vi "TestMethod.vi"() -> ()   [LabVIEW 2015]
panel:
  out "数据缓存":u8[](array[numeric])
  in  "停止":bool
  out "波形图":sgl[](graph)
  in  "读取方式":enum16{"bin", "csv"}(ring)
  in  "抓取波形数据指令集合":string(combo)="capture wave:.bin@CH:0@DT:vol;"
  out "Dll路径":path
  in  "超时(ms)":u32=2000
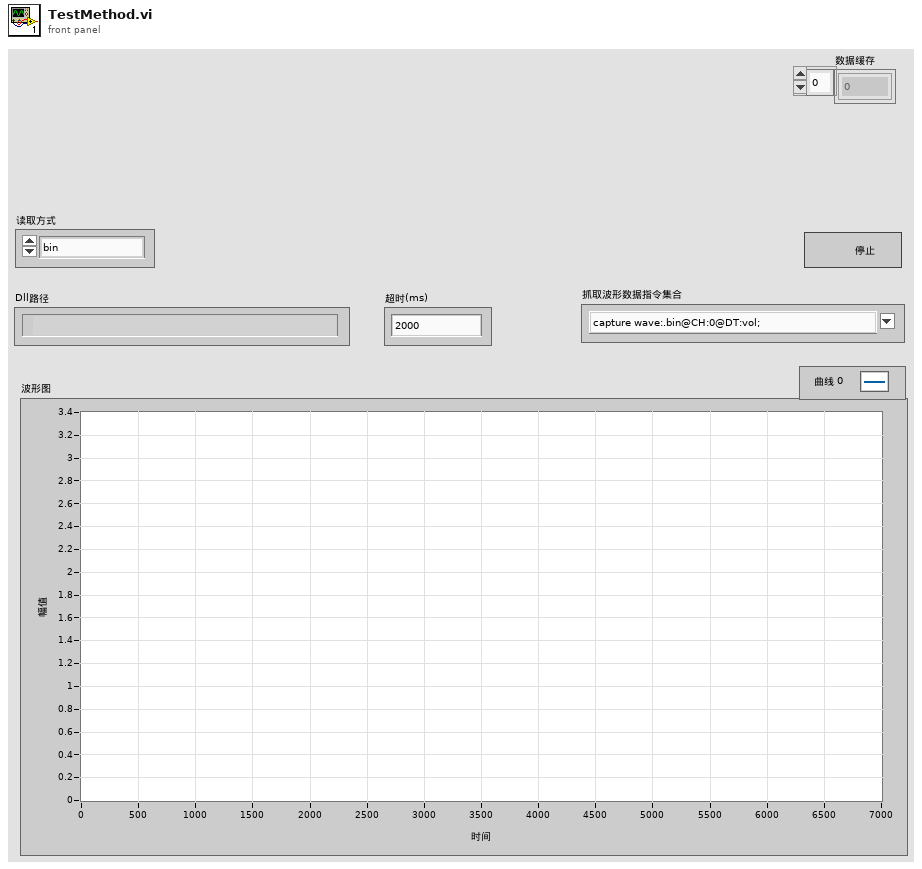
[diagram p1: front panel]
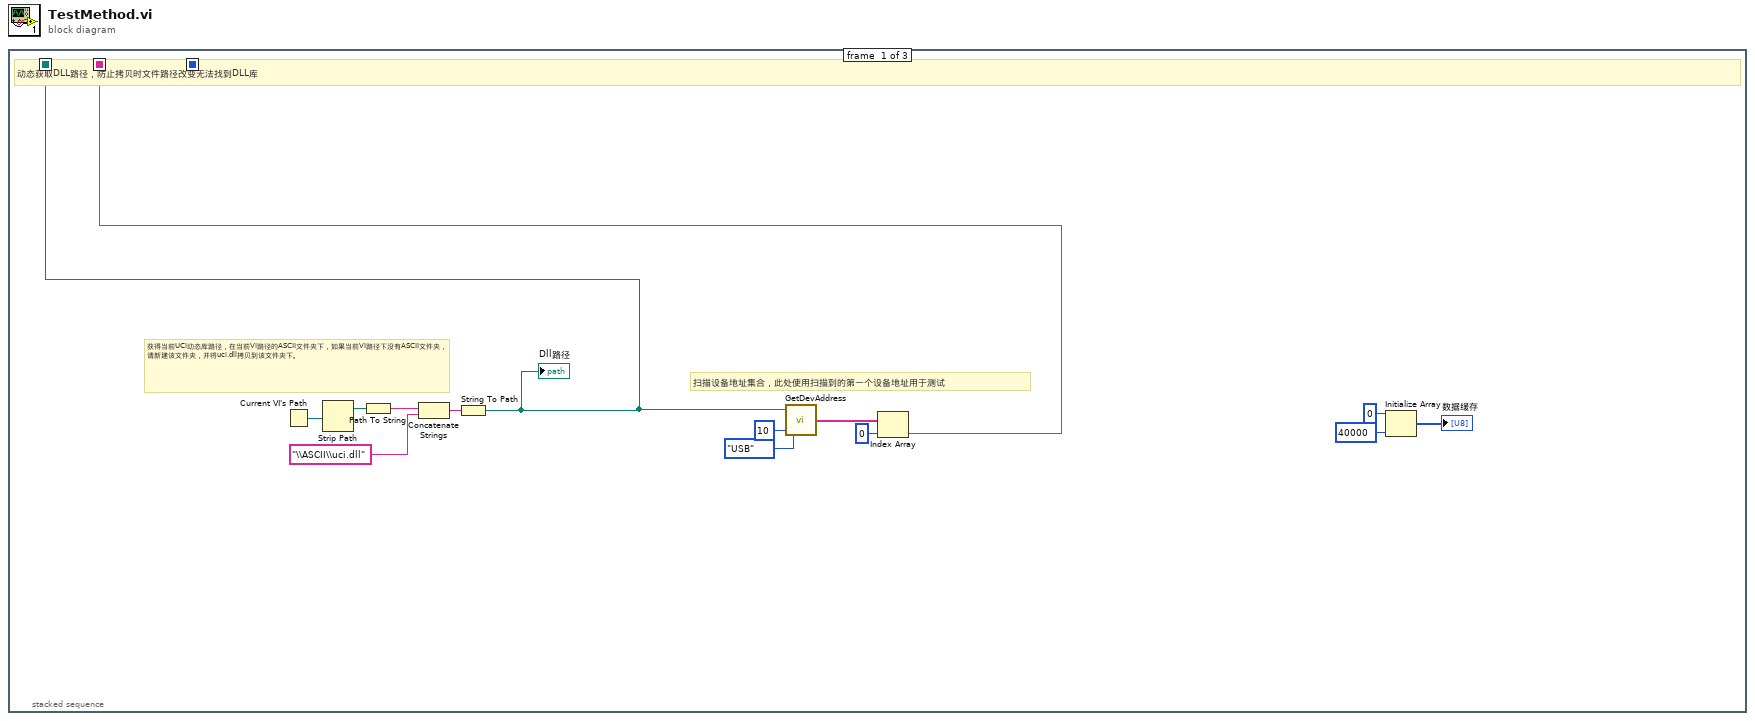
[diagram p0: block diagram]
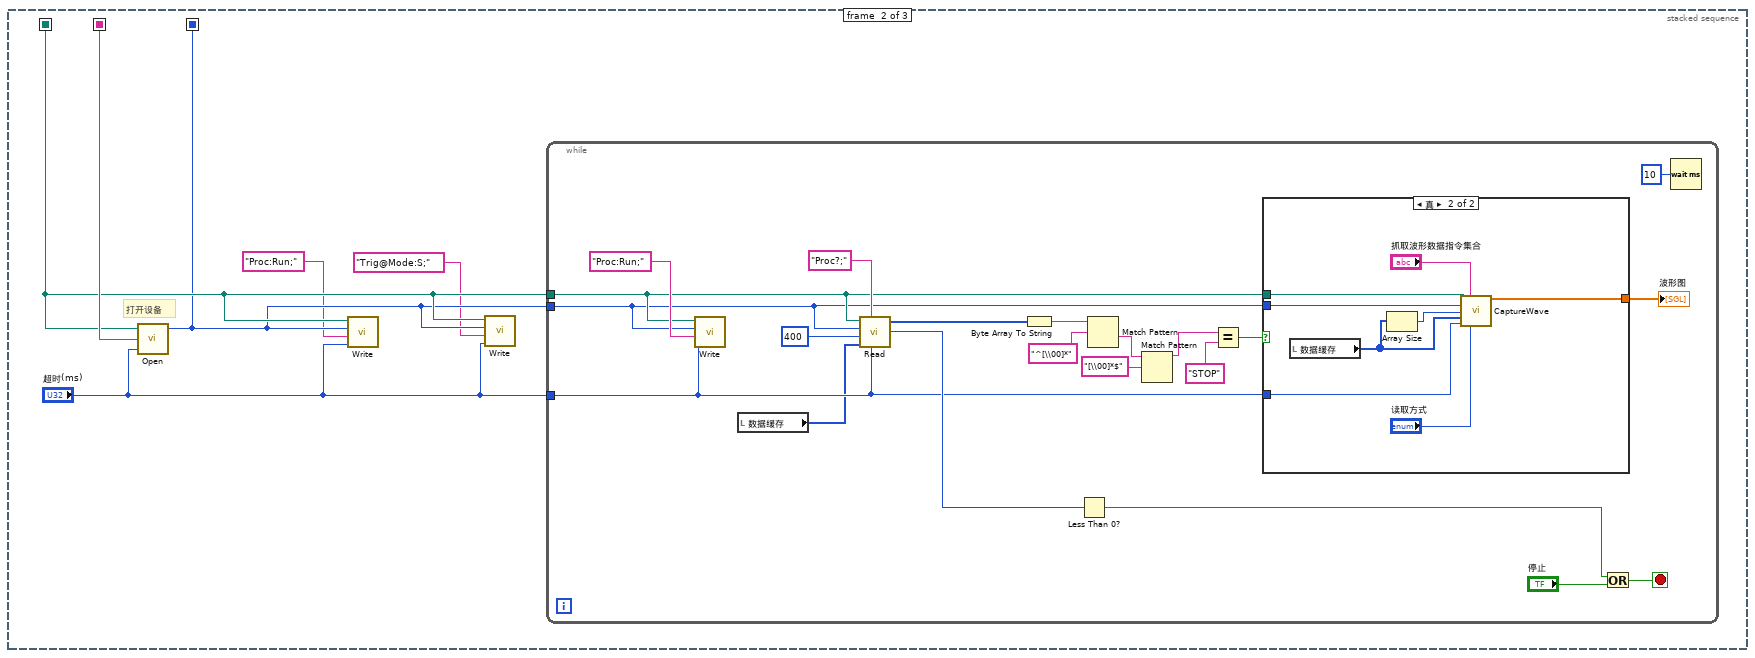
[diagram p2: hidden frame]
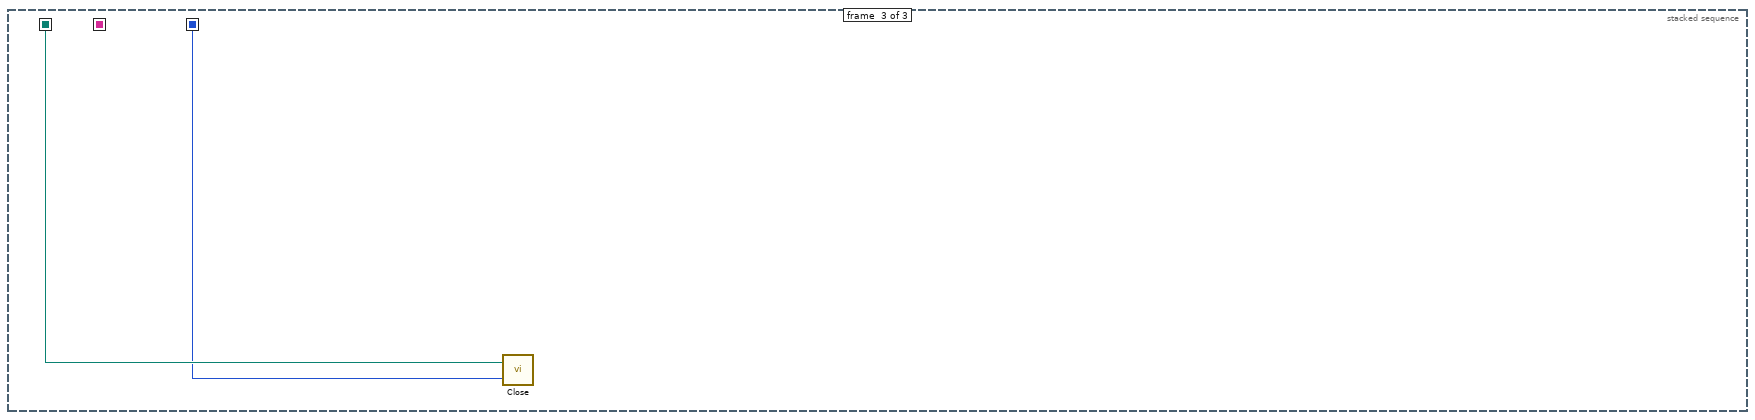
[diagram p4: hidden frame]
diagram:
  n1 = stacked-sequence {
    seq-local: [w9 _ _] -> [_ w19 w51]
    seq-local: [_ w18 _] -> [_ _ w50]
    seq-local: [w4 _ _] -> [_ w20 _]
    frame #0 {
      # "扫描设备地址集合，此处使用扫描到的第一个设备地址用于测试"
      # "获得当前UCI动态库路径，在当前VI路径的ASCII文件夹下，如果当前VI路径下没有ASCII文件夹，请新建该文件夹，并将uci.dll拷贝到该文件夹下。"
      # "动态获取DLL路径，防止拷贝时文件路径改变无法找到DLL库"
      n2 = Current VI's Path() -> (path=w13:path)
      n3 = Strip Path(path=w13) -> (stripped path=w11:path)  [unwired: 1 out]
      n4 = Path To String(path=w11) -> (string=w10:string)
      n5 = Concatenate Strings(w10, "\\ASCII\\uci.dll" ("字符串")) -> (w12:string)
      n6 = String To Path(string=w12) -> (path=w9:path)
      "Dll路径" <- w9
      n7 = call "GetDevAddress.vi"("DevNum"=u32 10 ("搜索设备数量"), "DevType"=enum16{"LAN", "USB"}."USB" ("设备类型"), "UCI_DllPath"=w9) -> ("DevAddressGroup"=w6:string[])
      n8 = Index Array(array=w6, index=0 ("索引")) -> (element=w4:string)
      n9 = Initialize Array(u8 0 ("元素"), 40000 ("维数大小")) -> (→"数据缓存":u8[])
    }
    frame #1 {
      # "打开设备"
      n10 = call "Open.vi"("Timeout"="超时(ms)", "Addr"=w20, "UCI_DllPath"=w19) -> ("Session_id"=w18:i32)  [unwired: 2 out]
      n11 = call "Write.vi"("UCI_DllPath"=w19, "Session_id"=w18, "Command"="Proc:Run;" ("指令"), "Timeout"="超时(ms)") -> ()  [unwired: 1 in, 1 out]
      n12 = call "Write.vi"("UCI_DllPath"=w19, "Session_id"=w18, "Command"="Trig@Mode:S;" ("指令"), "Timeout"="超时(ms)") -> ()  [unwired: 1 in, 1 out]
      n13 = while {
        tunnel: w19 -> [w29]
        tunnel: w18 -> [w27]
        tunnel: "超时(ms)" -> [w28]
        stop <- w24 stop-if-true
        n14 = call "Write.vi"("UCI_DllPath"=w29, "Session_id"=w27, "Command"="Proc:Run;" ("指令"), "Timeout"=w28) -> ()  [unwired: 1 in, 1 out]
        n15 = local read "数据缓存"() -> (w22:u8[])
        n16 = call "Read.vi"("UCI_DllPath"=w29, "Command"="Proc?;" ("指令"), "Session_id"=w27, "Length"=u32 400 ("len"), "Timeout"=w28, "InputData"=w22) -> ("OutputData"=w40:u8[], "Result"=w33:i32)  [unwired: 1 out]
        n17 = Byte Array To String(unsigned byte array=w40) -> (string=w34:string)
        n18 = Less Than 0?(x=w33) -> (x < 0?=w23:bool)
        n19 = Match Pattern(string=w34, regular expression="^[\\00]*") -> (after substring=w37:string)  [unwired: 1 in, 3 out]
        n20 = Match Pattern(string=w37, regular expression="[\\00]*$") -> (before substring=w31:string)  [unwired: 1 in, 3 out]
        n21 = Equal?(x=w31, y="STOP") -> (x = y?=w38:bool)
        n22 = case shown="真" w38 {
          tunnel: w29 -> [_ w47]
          tunnel: w27 -> [_ w48]
          tunnel: w28 -> [_ w46]
          tunnel: [_ w44] -> w26
          frame False {
          }
          frame True {
            n23 = local read "数据缓存"() -> (w42:u8[])
            n24 = Array Size(array=w42) -> (size(s)=w43:i32)
            n25 = call "CaptureWave.vi"("UCI_DllPath"=w47, "Command"="抓取波形数据指令集合", "Session_id"=w48, "Length"=w43, "InputData"=w42, "Timeout(ms)"=w46, "ReadType"="读取方式") -> ("OutputData"=w44:sgl[])  [unwired: 6 in, 2 out]
          }
        }
        "波形图" <- w26
        n26 = Or(x=w23, y="停止") -> (x .or. y?=w24:bool)
        n27 = Wait (ms)(milliseconds to wait=u32 10 ("等待时间（毫秒）")) -> ()  [unwired: 1 out]
      }
    }
    frame #2 {
      n28 = call "Close.vi"("Session_id"=w50, "UCI_DllPath"=w51) -> ()  [unwired: 1 out]
    }
  }
